vi "Handle Messages.vi"(8 "error in (no error)":errorcluster, 9 "Message Data":variant, 10 "Message":string, 11 "Application In":refnum<class "Application.lvclass">) -> (0 "error out":errorcluster, 3 "Application Out":refnum<class "Application.lvclass">)   [LabVIEW 2020, in "Application.lvclass"]
doc: "This is the main method handling incomming messages to the process. This method should be overridden to add functionality to the process or override functionality implemented by a parent. Any message not handled should be sent to the parent method using the default case. \nEach state should be atomic and states should not enqueue new messages from within this method. For cyclic iteration of an action, using a Helper Loop is recommended."
uses:
  Application.lvclass
  Application.lvclass/Application.ctl
  Process/Process.lvclass
  C:/git/astemes-triarc-framework/source/Framework/Process/Process.lvclass
  C:/git/astemes-triarc-framework/source/Framework/Async Handler/Async Handler.lvclass
  Async Handler/Async Handler.lvclass
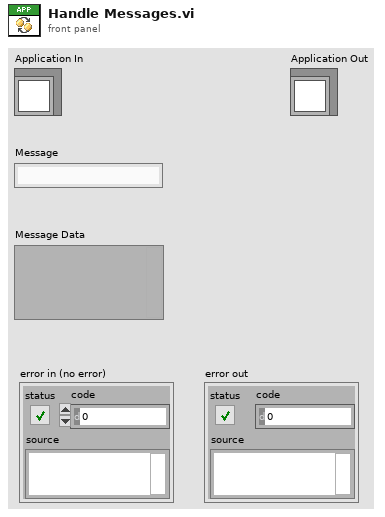
[diagram p1: front panel]
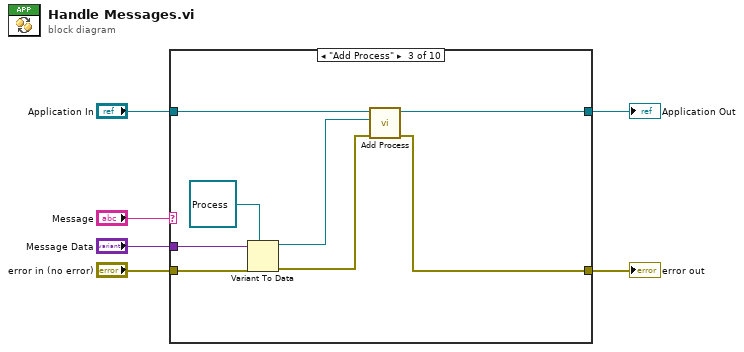
[diagram p0: block diagram]
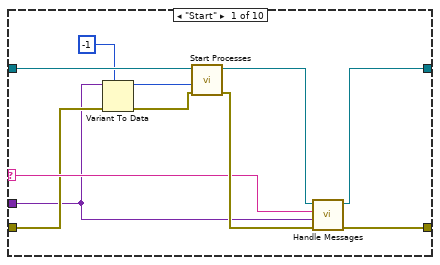
[diagram p2: hidden frame]
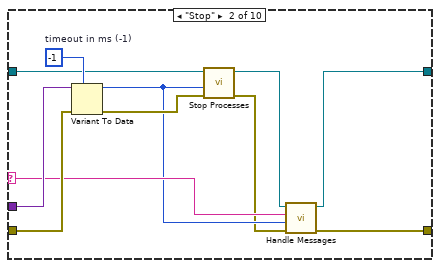
[diagram p3: hidden frame]
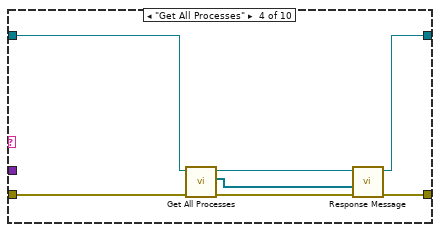
[diagram p4: hidden frame]
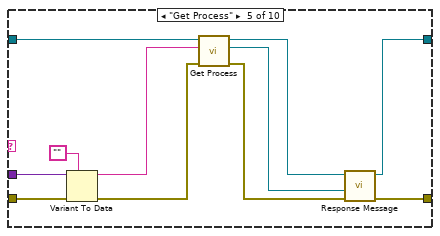
[diagram p5: hidden frame]
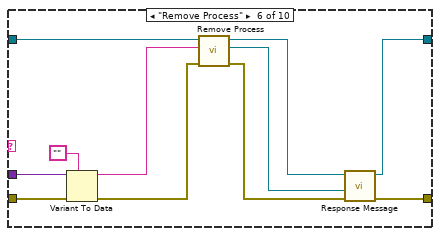
[diagram p6: hidden frame]
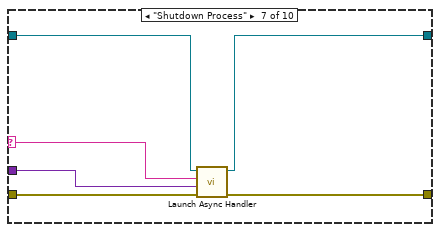
[diagram p7: hidden frame]
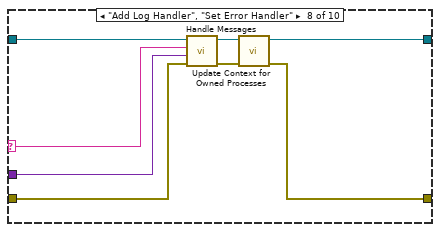
[diagram p8: hidden frame]
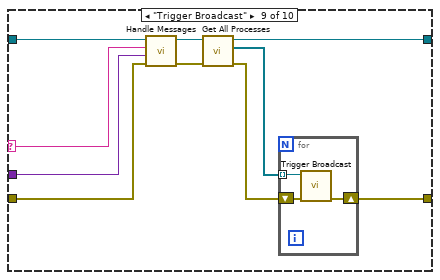
[diagram p9: hidden frame]
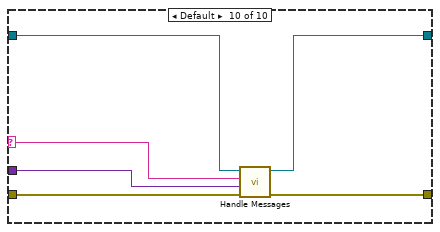
[diagram p10: hidden frame]
diagram:
  n1 = case shown="\"Add Process\"" "Message" {
    selector: "Message" -> [w14 w21 _ _ _ _ w68 w78 w86 w94]
    tunnel: [w16 w18 w34 w43 w53 w64 w70 w75 w80 w98] -> w6
    tunnel: [w13 w22 w29 w42 w52 w63 w69 w74 w84 w97] -> w1
    tunnel: "error in (no error)" -> [w11 w28 w35 w39 w54 w65 w71 w73 w87 w96]
    tunnel: "Message Data" -> [w7 w27 w36 _ w51 w62 w67 w77 w85 w95]
    tunnel: "Application In" -> [w12 w24 w30 w41 w48 w59 w66 w79 w89 w93]
    frame "Start" {
      n2 = Variant To Data(error in=w11, type=-1 ("Timeout [ms] (-1)"), Variant=w7) -> (data=w8:i32, error out=w10:errorcluster)
      n3 = call "Start Processes.vi"("error in (no error)"=w10, "Timeout [ms] (-1)"=w8, "Application In"=w12) -> ("error out"=w17:errorcluster, "Application Out"=w15:refnum<class "Application.lvclass">)  [unwired: 7 in]
      n4 = call-parent "Handle Messages.vi"("error in (no error)"=w17, "Message Data"=w7, "Message"=w14, "Process In"=w15) -> ("error out"=w16:errorcluster, "Process Out"=w13:refnum<class "Application.lvclass">)  [unwired: 6 in]
    }
    frame "Stop" {
      w26 = -1  # timeout in ms (-1)
      n5 = Variant To Data(error in=w28, type=w26, Variant=w27) -> (data=w20:i32, error out=w25:errorcluster)
      n6 = call "Stop Processes.vi"("error in (no error)"=w25, "timeout in ms (-1)"=w20, "Application In"=w24) -> ("error out"=w19:errorcluster, "Application Out"=w23:refnum<class "Application.lvclass">)  [unwired: 6 in, 1 out]
      n7 = call-parent "Handle Messages.vi"("error in (no error)"=w19, "Message Data"=w20, "Message"=w21, "Process In"=w23) -> ("error out"=w18:errorcluster, "Process Out"=w22:refnum<class "Application.lvclass">)  [unwired: 6 in]
    }
    frame "Add Process" {
      n8 = Variant To Data(error in=w35, type=refnum<class "Process.lvclass"> refnum ("Rig Process"), Variant=w36) -> (data=w32:refnum<class "Process.lvclass">, error out=w31:errorcluster)
      n9 = call "Add Process.vi"("error in (no error)"=w31, "Process"=w32, "Application In"=w30) -> ("error out"=w34:errorcluster, "Application Out"=w29:refnum<class "Application.lvclass">)  [unwired: 7 in]
    }
    frame "Get All Processes" {
      n10 = call "Get All Processes.vi"("error in (no error)"=w39, "Application In"=w41) -> ("error out"=w38:errorcluster, "App Processes"=w37:refnum<class "Process.lvclass">[], "Application Out"=w40:refnum<class "Application.lvclass">)  [unwired: 7 in]
      n11 = call "Response Message.vi"("error in (no error)"=w38, "Response Message Data"=w37, "Process In"=w40) -> ("error out"=w43:errorcluster, "Process Out"=w42:refnum<class "Application.lvclass">)  [unwired: 7 in]
    }
    frame "Get Process" {
      n12 = Variant To Data(error in=w54, type="", Variant=w51) -> (data=w46:string, error out=w45:errorcluster)
      n13 = call "Get Process.vi"("error in (no error)"=w45, "Process Name"=w46, "Application In"=w48) -> ("error out"=w44:errorcluster, "App Process"=w47:refnum<class "Process.lvclass">, "Application Out"=w49:refnum<class "Application.lvclass">)  [unwired: 6 in]
      n14 = call "Response Message.vi"("error in (no error)"=w44, "Response Message Data"=w47, "Process In"=w49) -> ("error out"=w53:errorcluster, "Process Out"=w52:refnum<class "Application.lvclass">)  [unwired: 7 in]
    }
    frame "Remove Process" {
      n15 = Variant To Data(error in=w65, type="", Variant=w62) -> (data=w57:string, error out=w56:errorcluster)
      n16 = call "Remove Process.vi"("error in (no error)"=w56, "Process Name"=w57, "Application In"=w59) -> ("error out"=w55:errorcluster, "App Process"=w58:refnum<class "Process.lvclass">, "Application Out"=w60:refnum<class "Application.lvclass">)  [unwired: 6 in]
      n17 = call "Response Message.vi"("error in (no error)"=w55, "Response Message Data"=w58, "Process In"=w60) -> ("error out"=w64:errorcluster, "Process Out"=w63:refnum<class "Application.lvclass">)  [unwired: 7 in]
    }
    frame "Shutdown Process" {
      n18 = call "Launch Async Handler.vi"("error in (no error)"=w71, "Message Data"=w67, "Message"=w68, "Async Action In"=w66) -> ("error out"=w70:errorcluster, "Async Action Out"=w69:refnum<class "Application.lvclass">)  [unwired: 6 in]
    }
    frame "Add Log Handler", "Set Error Handler" {
      n19 = call-parent "Handle Messages.vi"("error in (no error)"=w73, "Message Data"=w77, "Message"=w78, "Process In"=w79) -> ("error out"=w72:errorcluster, "Process Out"=w76:refnum<class "Application.lvclass">)  [unwired: 6 in]
      n20 = call "Update Context for Owned Processes.vi"("error in (no error)"=w72, "Application In"=w76) -> ("error out"=w75:errorcluster, "Application Out"=w74:refnum<class "Application.lvclass">)  [unwired: 8 in]
    }
    frame "Trigger Broadcast" {
      n21 = call-parent "Handle Messages.vi"("error in (no error)"=w87, "Message Data"=w85, "Message"=w86, "Process In"=w89) -> ("error out"=w83:errorcluster, "Process Out"=w88:refnum<class "Application.lvclass">)  [unwired: 6 in]
      n22 = call "Get All Processes.vi"("error in (no error)"=w83, "Application In"=w88) -> ("error out"=w81:errorcluster, "App Processes"=w82:refnum<class "Process.lvclass">[], "Application Out"=w84:refnum<class "Application.lvclass">)  [unwired: 7 in]
      n23 = for {
        tunnel: w82 -> [w92] mode=indexing
        shift-right: [w90] -> w80
        shift-left: w81 -> [w91]
        n24 = call "Trigger Broadcast.vi"("error in (no error)"=w91, "Process in"=w92) -> ("error out"=w90:errorcluster)  [unwired: 8 in, 1 out]
      }
    }
    frame Default {
      n25 = call-parent "Handle Messages.vi"("error in (no error)"=w96, "Message Data"=w95, "Message"=w94, "Process In"=w93) -> ("error out"=w98:errorcluster, "Process Out"=w97:refnum<class "Application.lvclass">)  [unwired: 6 in]
    }
  }
  "error out" <- w6
  "Application Out" <- w1
